vi "Own20261012_PublicGetCaseSelectorSides_v2.vi"() -> ()   [LabVIEW 2024]
panel:
  out "error out":errorcluster caption="错误输出"
  out "outside_id":refnum<vi>
  out "inside_ids":refnum<vi>[](array[refnum])
  out "tunnel_id":refnum<vi>
  in  "case_id":u32
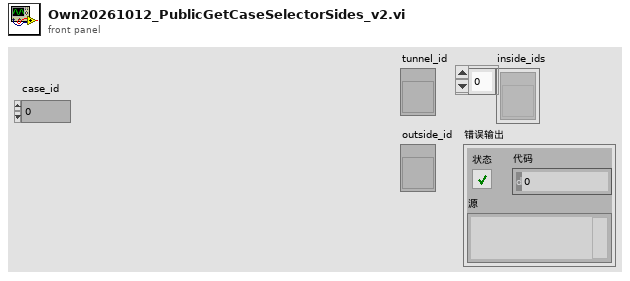
[diagram p1: front panel]
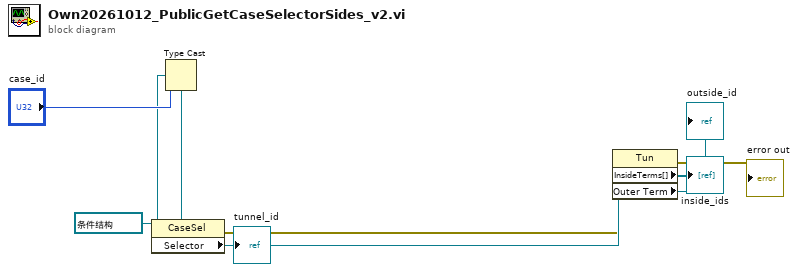
[diagram p0: block diagram]
diagram:
  n1 = Type Cast(type=refnum<vi> refnum ("引用"), x="case_id") -> (*(type *) &x=w6:refnum<vi>)
  n2 = property on="属性节点" class="CaseSel"(reference=w6) -> (error out=w4:errorcluster, "Selector"=w5:refnum<vi>)  [unwired: 1 in, 1 out]
  "tunnel_id" <- w5
  n3 = property class="Tun"(reference=w5, error in=w4) -> (error out=→"error out":errorcluster, "InsideTerms[]"=→"inside_ids":refnum<vi>[], "Outer Term"=→"outside_id":refnum<vi>)  [unwired: 1 out]
